vi "set Marker X Position Frequency.vi"(8 "error in (no error)":errorcluster, 9 "Index":i32, 10 "X Position Frequency (Hz)":dbl, 11 "FSV-40N in":refnum<class "FSV-40N.lvclass">) -> (0 "error out":errorcluster, 3 "FSV-40N out":refnum<class "FSV-40N.lvclass">)   [LabVIEW 2023, in "Spectrum Analyzer.lvlib" / "FSV-40N.lvclass"]
uses:
  FSV-40N.lvclass
  TYPE DEFINITION/TYPE Marker Control Mode.ctl
  FSV-40N.lvclass/FSV-40N.ctl
  Spectrum Analyzer.lvlib
  <vilib>/ErrorRing/Error Ring.xnode
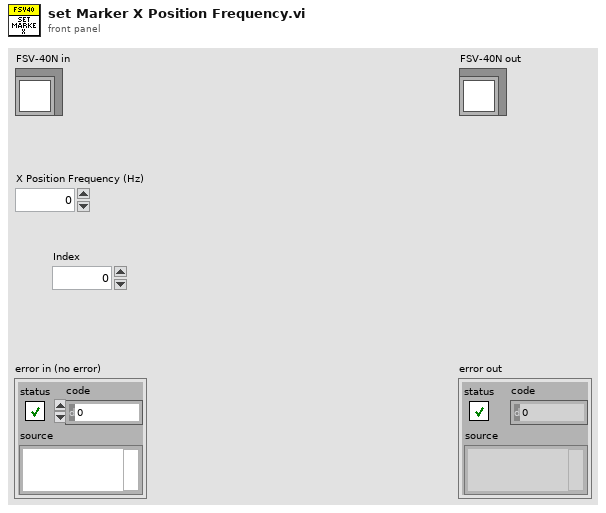
[diagram p1: front panel]
types:
  T1 = typedef "Spectrum Analyzer.lvlib/TYPE Marker Control Mode.ctl" = enum16{"Normal", "Delta", "Off"}
  T2 = typedef "Spectrum Analyzer.lvlib/TYPE Marker Type Map.ctl" = map{i32, T1}
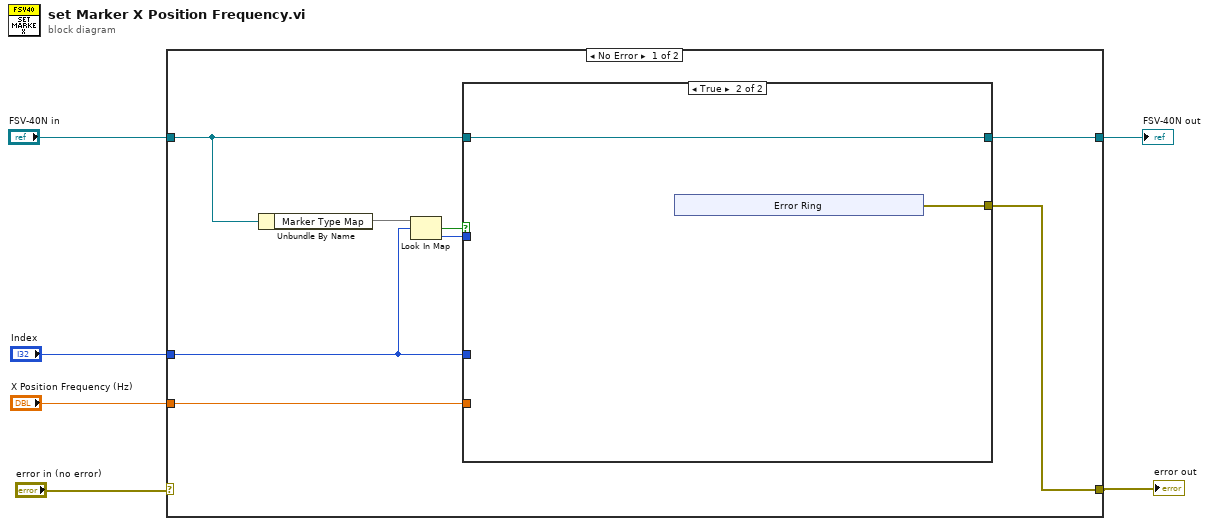
[diagram p0: block diagram]
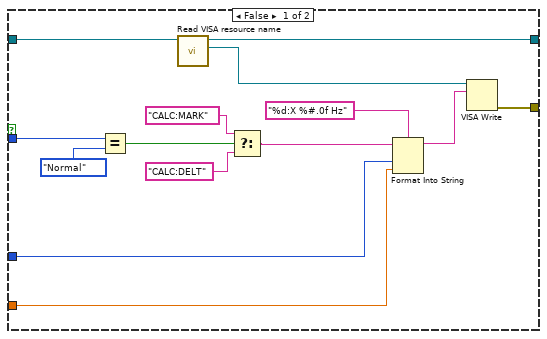
[diagram p2: hidden frame]
diagram:
  n1 = case shown="No Error" "error in (no error)" {
    selector: "error in (no error)" -> [_ w32]
    tunnel: "FSV-40N in" -> [w11 w33]
    tunnel: [w14 w33] -> w5
    tunnel: [w12 w32] -> w3
    tunnel: "Index" -> [w9 _]
    tunnel: "X Position Frequency (Hz)" -> [w13 _]
    frame No Error {
      n2 = Unbundle By Name(w11) -> ("Marker Type Map"=w10:T2)
      n3 = Look In Map(map=w10, key=w9) -> (key not found?=w7:bool, value=w8:T1)  [unwired: 1 in]
      n4 = case shown="True" w7 {
        tunnel: [w27 w30] -> w14
        tunnel: w13 -> [w25 _]
        tunnel: [w23 w29] -> w12
        tunnel: w11 -> [w22 w30]
        tunnel: w9 -> [w21 _]
        tunnel: w8 -> [w20 _]
        frame False {
          n5 = Equal?(x=w20, y=TYPE_Marker_Control_Mode."Normal") -> (x = y?=w18:bool)
          n6 = call "Read VISA resource name.vi"("FSV-40N in"=w22) -> ("VISA resource name"=w28:refnum<visa-resource-name>, "FSV-40N out"=w27:refnum<class "FSV-40N.lvclass">)  [unwired: 8 in, 1 out]
          n7 = Select(t="CALC:MARK" ("initial string"), s=w18, f="CALC:DELT" ("initial string")) -> (s? t:f=w15:string)
          n8 = Format Into String(format string="%d:X %#.0f Hz", initial string=w15, w21, w25) -> (resulting string=w24:string)  [unwired: 1 in, 1 out]
          n9 = VISA Write(VISA resource name=w28, write buffer=w24) -> (error out=w23:errorcluster)  [unwired: 1 in, 2 out]
        }
        frame True {
          n10 = xnode "Error Ring"() -> ("error out"=w29:errorcluster)
        }
      }
    }
    frame Error {
    }
  }
  "error out" <- w3
  "FSV-40N out" <- w5
